vi "Main.vi"() -> ()   [LabVIEW 2013]
doc: "This template is for the Queued Message Handler design pattern.\n\nThe Event Handling Loop generates messages based on user interface actions.\n\nThe Message Handling Loop processes messages generated by the Event Handling Loop, or by other messages. The messages are string values, so new messages can be added easily to the Message Cases case structure in the Message Handling Loop. Each message cluster can also provide an optional value for Message Data, which is a variant that can be converted to whatever message-specific data is required."
uses:
  <vilib>/vision/Image Controls.llb/IMAQ Image.ctl
  Image Processing/Mask ROI FG Enum.ctl
  Message Passing/MsgQ Loops enum.ctl
  System Status/Status FG Enum.ctl
  Globals/Average Sector Data.vi
  controls/UI Data.ctl
  Message Queue/Message Queue.lvlib
  User Event - Stop/User Event - Stop.lvlib
  FPGA/FPGA Frame Grabbing.lvlib
  Image Processing/Image Processing.lvlib
  Common/State Machines/State Machine Lib.lvlib
  Message Passing/Main MsgQ.lvlib
  Common/GUI/GUI.lvlib
  <vilib>/rvi/interface/nirviReadWriteControl/nirviReadWriteControl.xnode
  FGs/FPGA_Reference.ctl
  FPGA Bitfiles/Simulation_WBA.lvbitx
  <vilib>/rvi/errors/niLvFpgaMergeErrorWithErrorCode.vi
  NiFpgaLv.dll
  <vilib>/rvi/errors/niLvFpgaAdjustHostInterfaceError.vi
panel:
  out "Frame Count":u16
  out "Frames Acquired":u32
  in  "Disable Background Subtraction":bool
  out "Analysis Ticks":u32
  out "Accumulate Ticks":u32
  out "FPGA Display Image":T1(plugin-control)
  out "Right Wingbeat Avg Graph":u8[](graph)
  in  "Start Serial Server":bool=TRUE
  out "Left Wingbeat Avg Graph":u8[](graph)
  in  "Stop Charts":bool
  in  "Wing ROIs":T2
  out "FPGA image info":T5={"Image Type"=0, "Unit"=enum."Undefined", "X Resolution"=2040, "Y Resolution"=1088, "X Step"=1.0, "Y Step"=1.0, "Image Name"="Image"} {"Image Type" items=["Grayscale (U8)", "Grayscale (I16)", "Grayscale (SGL)", "Complex (CSG)", "RGB (U32)", "HSL (U32)", "RGB (U64)", "Grayscale (U16)"]}
  in  "Stream?":bool
  out "FPGA Image":T1
  in  "Test Visual Response":bool
  in  "Test FPGA":bool
  out "Status Update":string="VI Stopped"
  in  "Define Mask":bool
  in  "Acquire Image":bool
  in  "Stop":bool
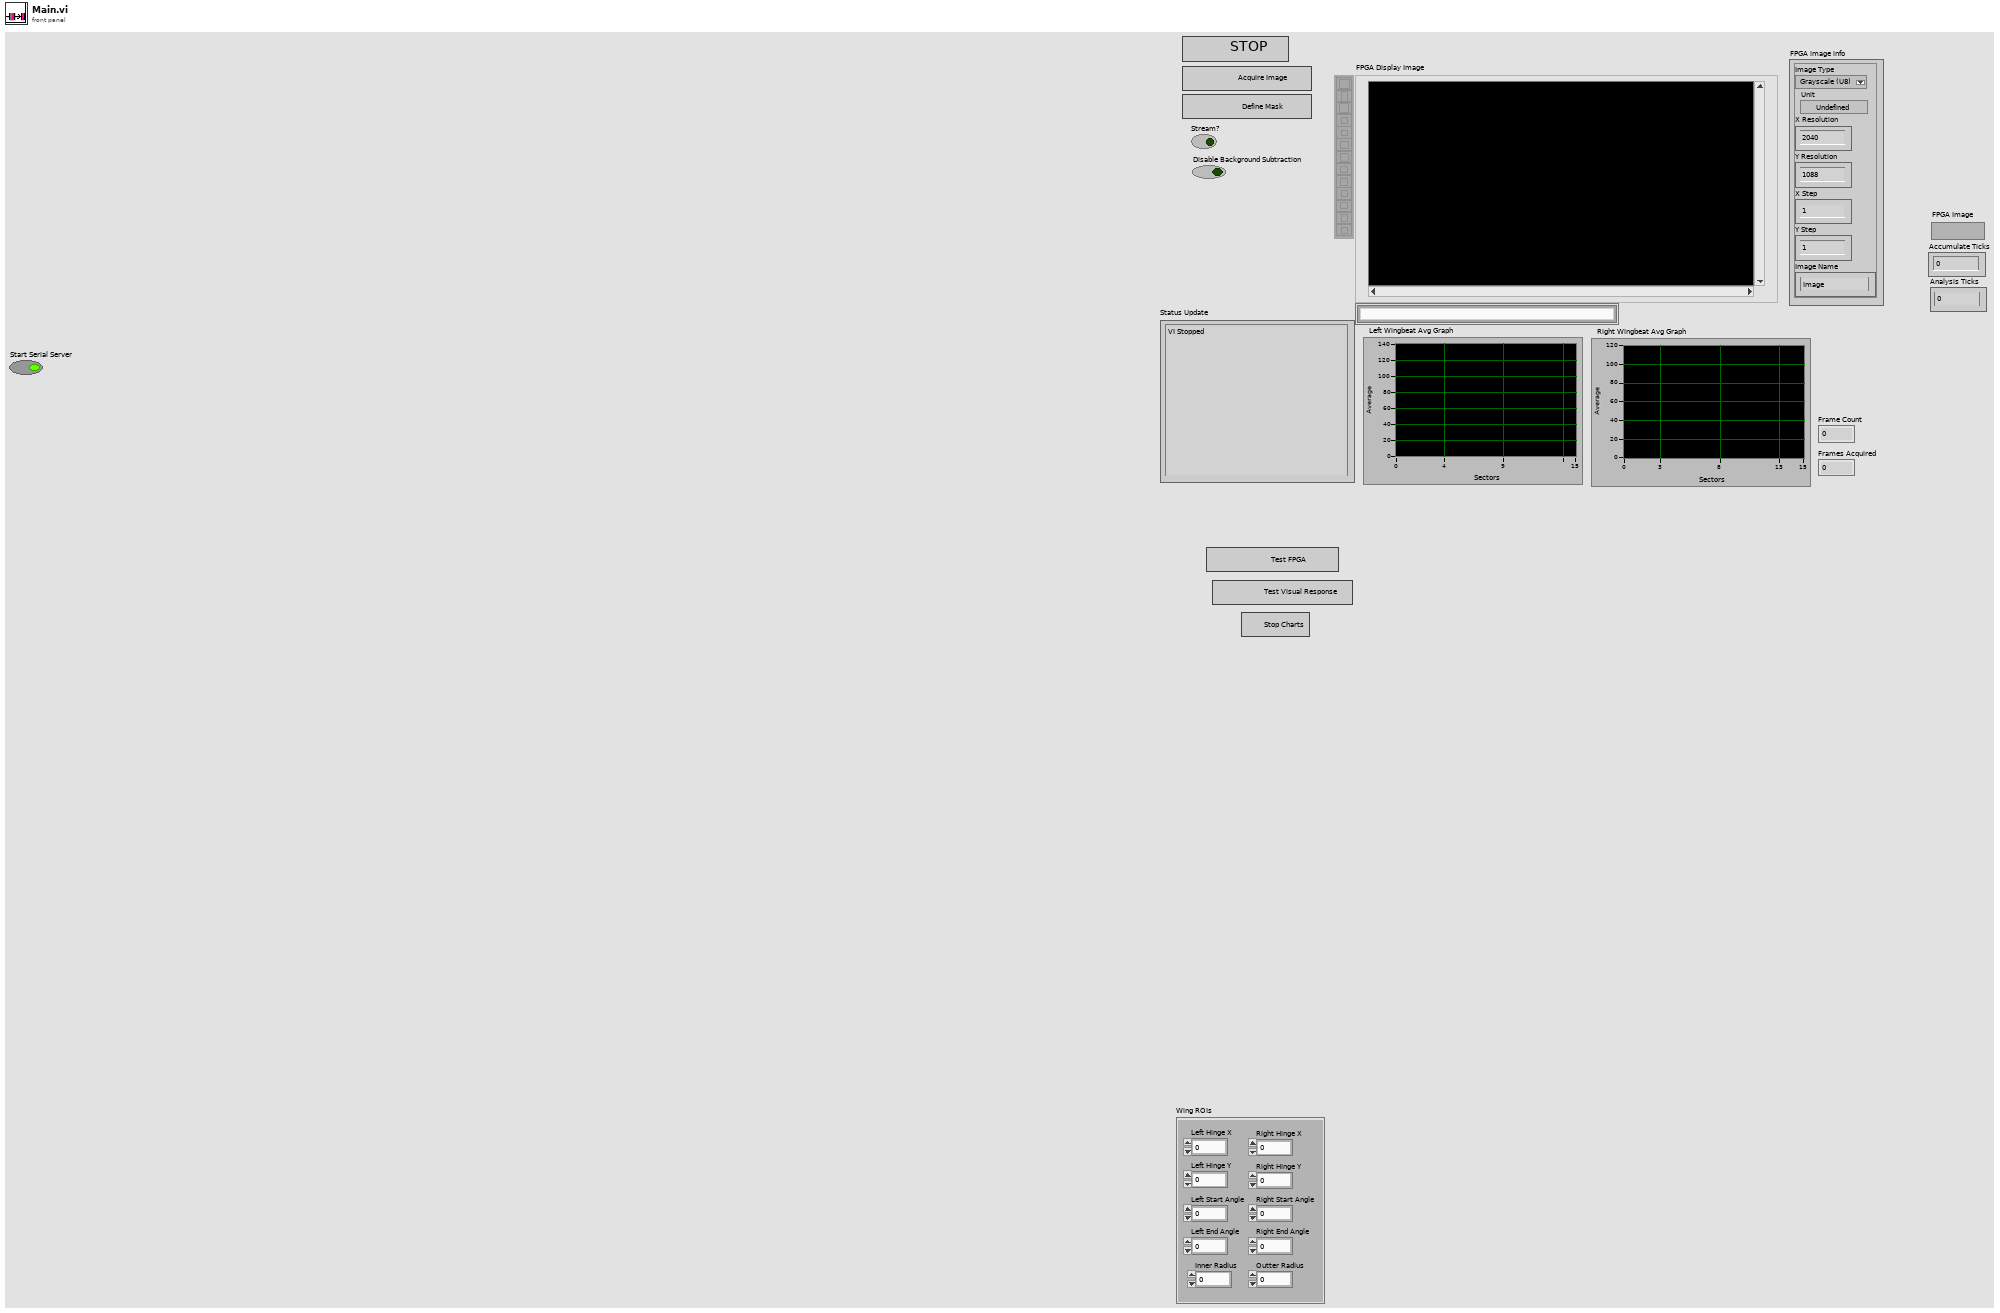
[diagram p1: front panel]
types:
  T1 = typedef "IMAQ Image.ctl" = refnum<image>
  T2 = cluster{"Left Hinge X":u16, "Left Hinge Y":u16, "Inner Radius":u16, "Outter Radius":u16, "Right Hinge X":u16, "Right Hinge Y":u16, "Right Start Angle":i16, "Right End Angle":i16, "Left Start Angle":i16, "Left End Angle":i16}
  T3 = typedef "Image Type" = u32
  T4 = typedef "Image Unit" = enum32{"Undefined", "Angström", "Micrometer", "Millimeter", "Centimeter", "Meter", "Kilometer", "Microinch", "Inch", "Feet", "Nautical miles", "Standard miles", "Steps"}
  T5 = cluster{"Image Type":T3, "Unit":T4, "X Resolution":i32, "Y Resolution":i32, "X Step":sgl, "Y Step":sgl, "Image Name":string}
  T6 = typedef "State Machine Lib.lvlib/STATE cluster.ctl" = cluster{"State":string, "Parameters":variant}
  T7 = typedef "Main MsgQ.lvlib/MsgQ Loops enum.ctl" = enum16{"User Interface", "Image Acq"}
  T8 = typedef "Mask ROI FG Enum.ctl" = enum16{"Read", "Write", "Enable Background", "Disable Background"}
  T9 = typedef "Status FG Enum.ctl" = enum16{"Reset", "Read", "Write"}
  T10 = typedef "FPGA_Reference.ctl" = refnum<k20>
  T11 = typedef "Mask ROI Cluster.ctl" = cluster{"left annulus":T12, "right annulus":T12, "Threshold Range":cluster{"Lower value":dbl, "Upper value":dbl}, "[Avg BG]":u8[], "Number of Sectors":u8, "Left ROI":T13, "Right ROI":T13, "Left Start Angle Duty Cycle":fxp<+,8,0>, "Left End Angle Duty Cycle":fxp<+,8,0>, "Right End Angle Duty Cycle":fxp<+,8,0>, "Right Start Angle Duty Cycle":fxp<+,8,0>, "[Sector ROIs]":T13[]}
  T12 = typedef "IMAQ Circle" = cluster{"Center X":i32, "Center Y":i32, "Inner Radius":i32, "Outer Radius":i32, "Start Angle":dbl, "End Angle":dbl}
  T13 = typedef "ROI Descriptor" = cluster{"Global Rectangle":i32[], "Contours":cluster{"ID":enum32{"External", "Internal"}, "Type":u32, "Coordinates":i32[]}[]}
  T14 = typedef "UI Data.ctl" = cluster{"Boolean <Replace Me>":bool, "Initial Message":string, "Numeric <Replace Me>":dbl, "Acquire Image Ref":refnum<vi>, "Define Mask Ref":refnum<vi>, "Status Update Ref":refnum<vi>, "Stop Button Ref":refnum<vi>, "FPGA Image":T1, "Processed Image":T1, "Left Annulus":cluster{"Center X":i32, "Center Y":i32, "Inner Radius":i32, "Outer Radius":i32, "Start Angle":dbl, "End Angle":dbl}, "Right Annulus":cluster{"Center X":i32, "Center Y":i32, "Inner Radius":i32, "Outer Radius":i32, "Start Angle":dbl, "End Angle":dbl}}
  T15 = typedef "Message Queue.lvlib/All Message Queues.ctl" = cluster{"UI":refnum<queue>}
  T16 = cluster{"Center X":i32, "Center Y":i32, "Inner Radius":i32, "Outer Radius":i32, "Start Angle":dbl, "End Angle":dbl}
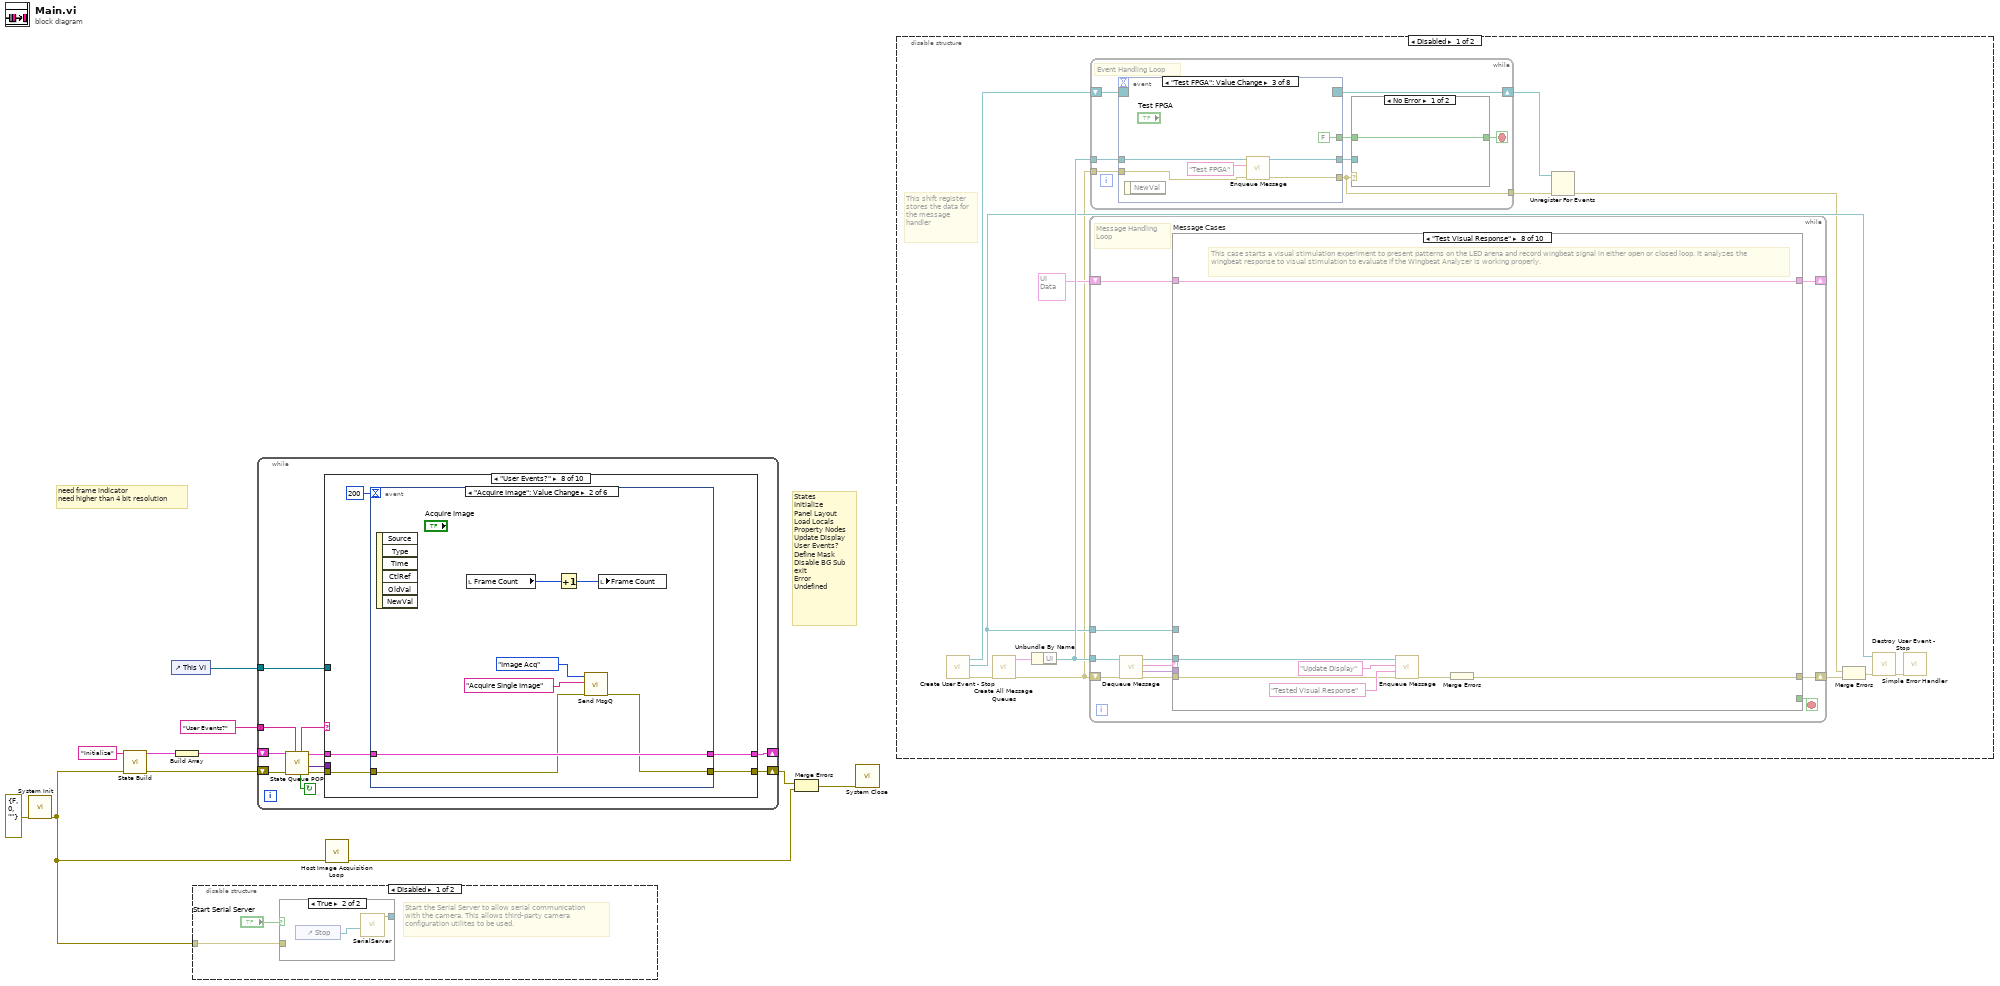
[diagram p0: block diagram]
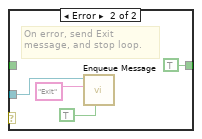
[diagram p4: hidden frame]
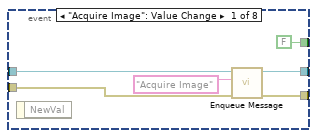
[diagram p5: hidden frame]
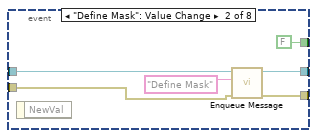
[diagram p6: hidden frame]
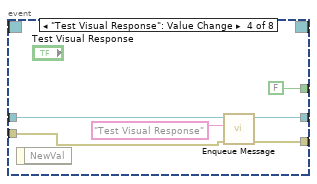
[diagram p7: hidden frame]
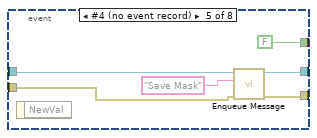
[diagram p8: hidden frame]
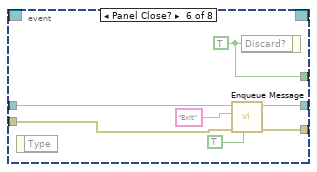
[diagram p9: hidden frame]
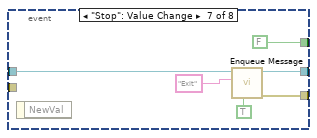
[diagram p10: hidden frame]
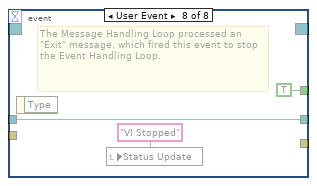
[diagram p11: hidden frame]
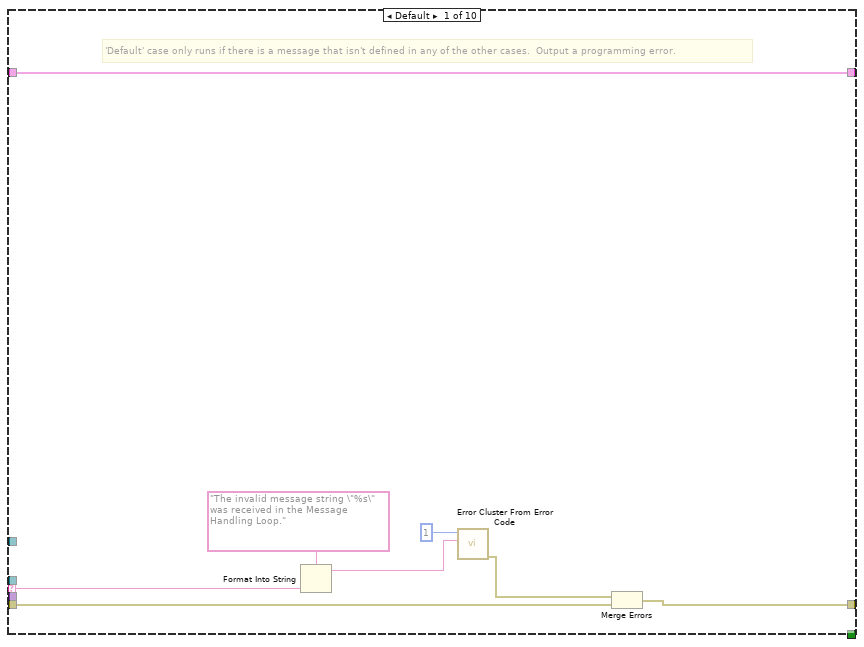
[diagram p12: hidden frame]
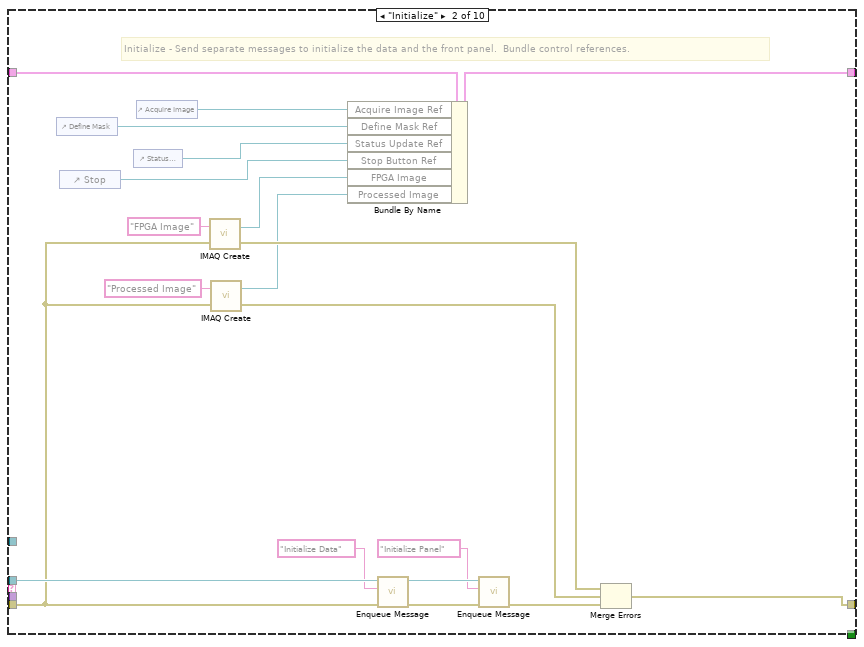
[diagram p13: hidden frame]
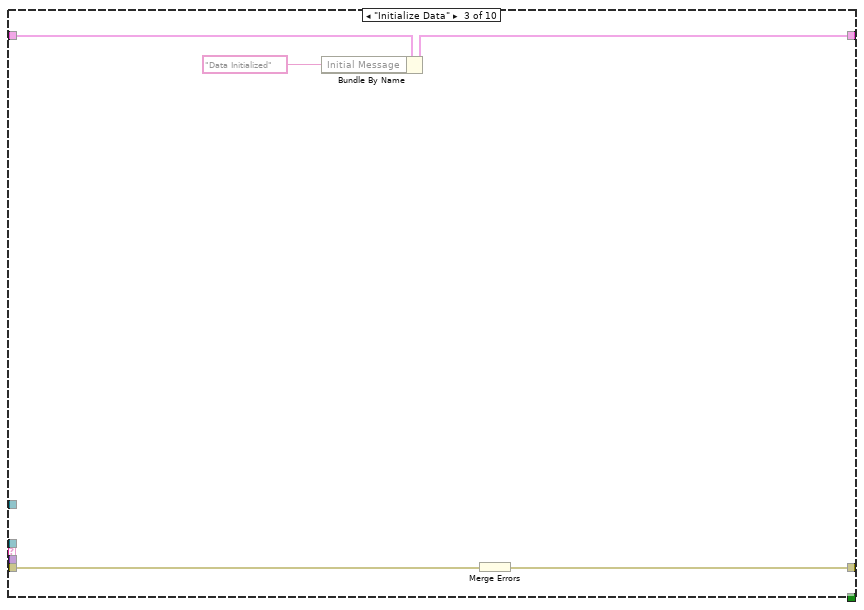
[diagram p14: hidden frame]
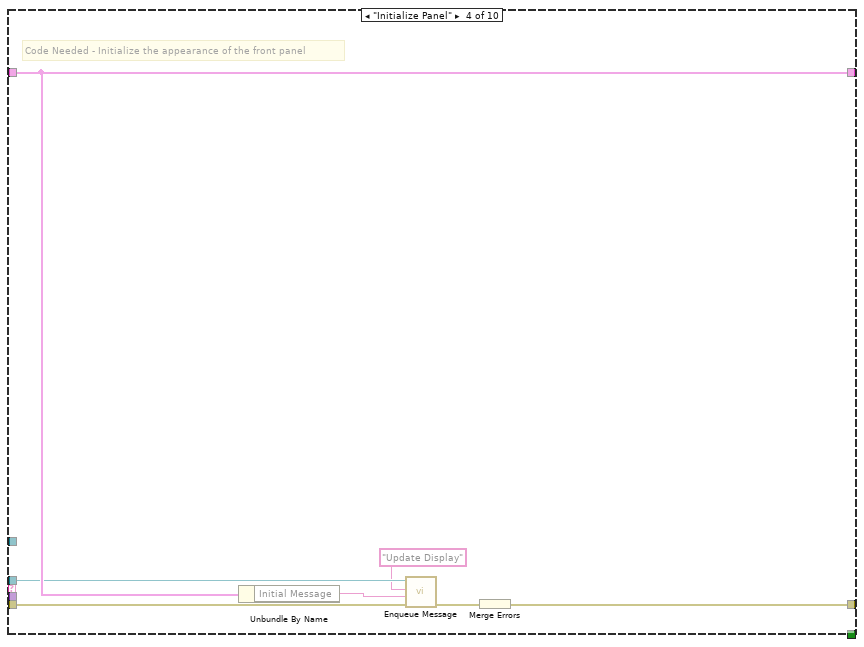
[diagram p15: hidden frame]
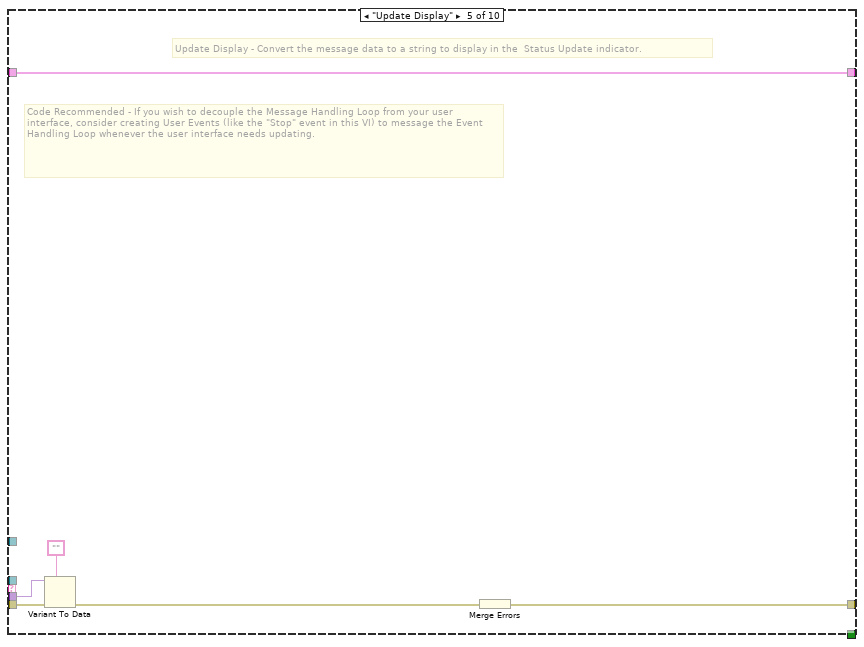
[diagram p16: hidden frame]
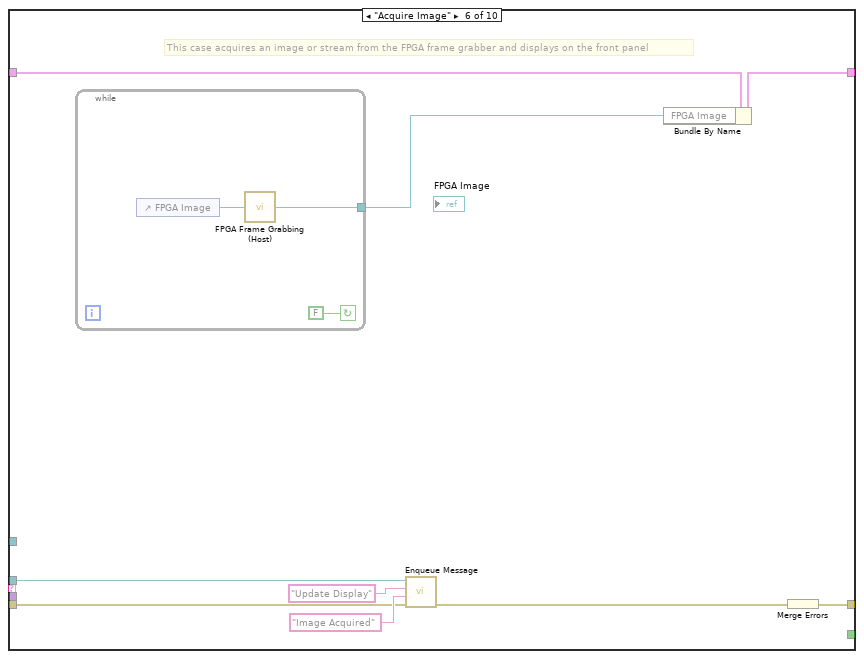
[diagram p17: hidden frame]
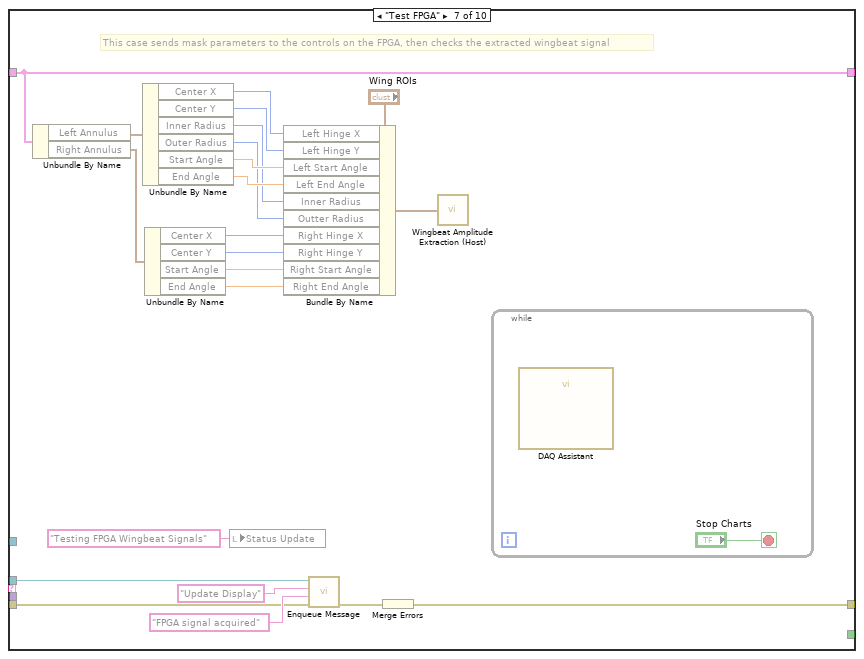
[diagram p18: hidden frame]
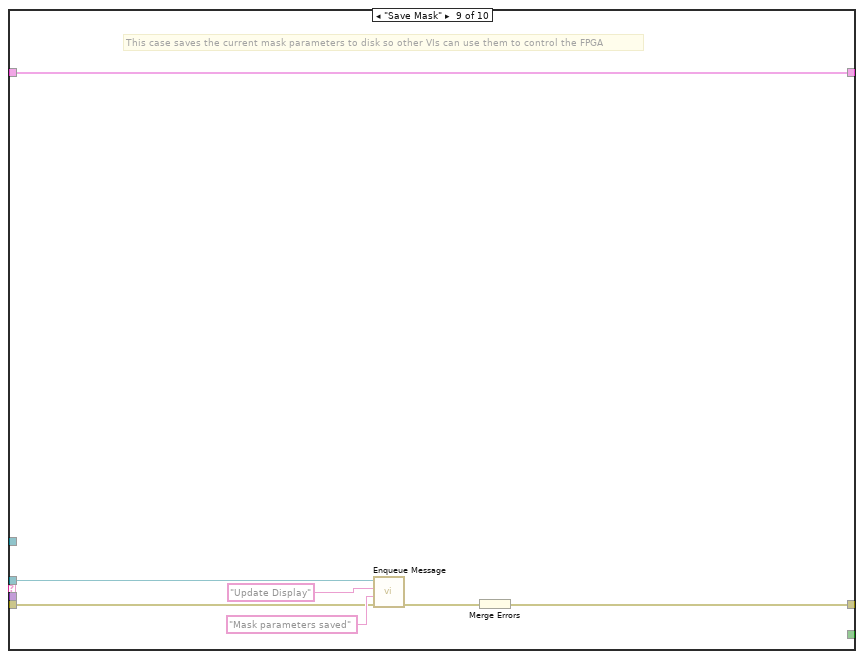
[diagram p19: hidden frame]
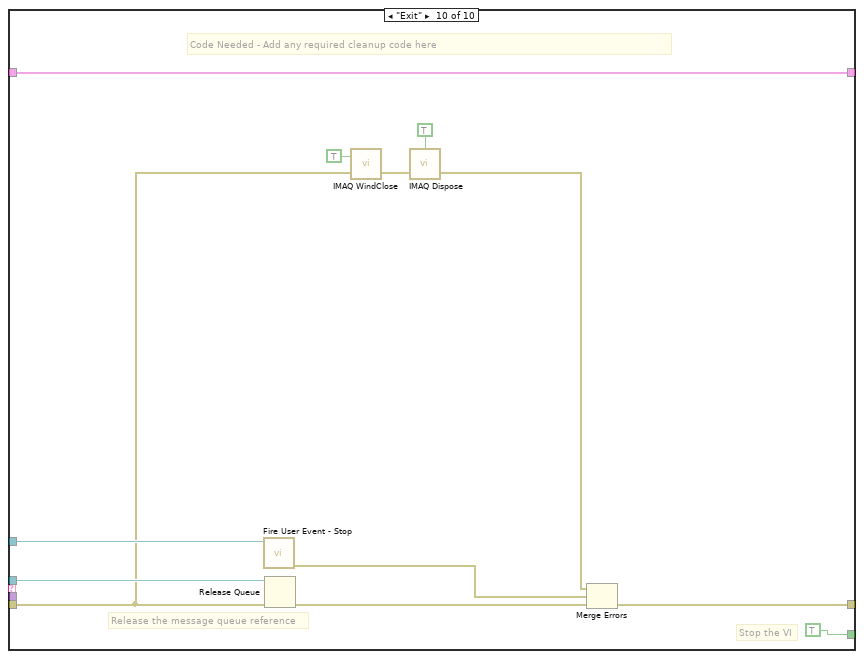
[diagram p20: hidden frame]
diagram:
  # "need frame indicator\nneed higher than 4 bit resolution"
  # "States\nInitialize\nPanel Layout\nLoad Locals\nProperty Nodes\nUpdate Display\nUser Events?\nDefine Mask\nDisable BG Sub\nexit\nError\nUndefined"
  n1 = call "System Init.vi"("error in (no error)"=errorcluster {"status"=FALSE, "code"=0, "source"=""}) -> ("error out"=w10:errorcluster)  [unwired: 10 in]
  n2 = call "State Build.vi"("error in (no error)"=w10, "State"="Initialize") -> ("error out"=w6:errorcluster, "State Out"=w8:T6)  [unwired: 8 in]
  n3 = control-ref of="This VI"() -> (w4:refnum<vi>)
  n4 = Build Array(w8) -> (w7:T6[])
  n5 = disable-structure shown="Disabled" {
    disable-tunnel: w10 -> [w12 _]
    frame Disabled {
      # "Start the Serial Server to allow serial communication\nwith the camera. This allows third-party camera\nconfiguration utilites to be used."
      n6 = case shown="True" "Start Serial Server" {
        tunnel: [_ w15] -> _
        tunnel: w12 -> [_ _]
        frame False {
        }
        frame True {
          n7 = control-ref of="Stop"() -> (w14:refnum<vi>)
          n8 = call "SerialServer.vi"("Stop Refnum"=w14) -> ("FPGA VI Reference Out"=w15:refnum<k20>)  [unwired: 6 in]
        }
      }
    }
    frame Enabled {
    }
  }
  n9 = while {
    shift-right: [w20] -> _
    shift-left: w7 -> [w26]
    shift-right: [w18] -> w3
    shift-left: w6 -> [w25]
    tunnel: "User Events?" ("State") -> [w23]
    tunnel: w4 -> [w21]
    stop <- w24 continue-if-true
    n10 = call "State Queue POP.vi"("Default state"=w23, "error in (no error)"=w25, "State que in"=w26) -> ("error out"=w17:errorcluster, "Parameters"=w16:variant, "State que out"=w19:T6[], "Not Exit?"=w24:bool, "State case out"=w22:string)  [unwired: 4 in]
    n11 = case shown="\"User Events?\"" w22 {
      tunnel: w21 -> [_ _ w37 _ _ _ _ _ _ _]
      tunnel: [w28 w29 w34 w41 w43 w48 w49 w65 w105 w133] -> w20
      tunnel: w19 -> [w28 w32 w34 w41 w43 w48 w49 w64 _ w133]
      tunnel: [w27 w30 w35 w40 w42 w46 w50 w63 w104 w131] -> w18
      tunnel: w17 -> [w27 w31 w36 w40 w42 w47 w51 w62 w106 w115]
      tunnel: w16 -> [_ _ _ _ _ _ w52 _ _ _]
      frame Default {
      }
      frame "Initialize" {
        n12 = call "State Queue PUSH multiple states no parameters.vi"("States to queue"=string[] ["Panel Layout", "Load Locals", "Property Nodes", "Update Display"], "error in (no error)"=w31, "State que in"=w32) -> ("error out"=w30:errorcluster, "State que out"=w29:T6[])  [unwired: 7 in]
      }
      frame "Panel Layout" {
        # "Reset origin to 0,0"
        n13 = call "Reset all pane origins.vi"("error in (no error"=w36, "Vi Ref In"=w37) -> ("error out"=w35:errorcluster)  [unwired: 8 in, 1 out]
      }
      frame "Load Locals" {
        w39 = FALSE ("Stream?")
        n14 = local write "Stream?"(w39) -> ()
        n15 = local write "Disable Background Subtraction"(w39) -> ()
        "Frame Count" <- u16 0 ("Frame Count")
      }
      frame "Property Nodes" {
      }
      frame "Define Mask" {
        n16 = call "Image References.vi"() -> ("Images"=w44:cluster{"Acquired Image":T1, "Display Image":T1})  [unwired: 10 in, 1 out]
        n17 = Unbundle By Name(w44) -> ("Acquired Image"=w45:T1)
        n18 = call "Define Mask.vi"("error in (no error)"=w47, "FPGA Image"=w45) -> ("error out"=w46:errorcluster)  [unwired: 9 in]
      }
      frame "Disable BG Sub" {
        n19 = Variant To Data(error in=w51, type=FALSE, Variant=w52) -> (data=w60:bool, error out=w57:errorcluster)
        n20 = Select(t=Mask_ROI_FG_Enum."Disable Background" ("Operation"), s=w60, f=Mask_ROI_FG_Enum."Enable Background" ("Operation")) -> (s? t:f=w56:T8)
        n21 = call "Mask ROI FG.vi"("error in (no error)"=w57, "Operation"=w56) -> ("error out"=w53:errorcluster)  [unwired: 8 in, 1 out]
        n22 = call "Send MsgQ.vi"("error in (no error)"=w53, "Message String"="Update Sector Parameters", "Send to MsgQ"=MsgQ_Loops_enum."Image Acq") -> ("error out"=w50:errorcluster)  [unwired: 8 in]
      }
      frame "User Events?" {
        n23 = event shown="[1] \"Acquire Image\": Value Change" {
          selector: _ -> [_ _ _ _ _ _]
          dyn-events: _ -> [_ _ _ _ _ _]
          timeout: 200 -> [_ _ _ _ _ _]
          tunnel: [w68 w80 w83 w90 w96 w99] -> w65
          tunnel: w64 -> [w69 w80 w83 w92 w97 w102]
          tunnel: [w70 w77 w84 w89 w95 w100] -> w63
          tunnel: w62 -> [w71 w78 w85 w91 w94 w101]
          event Timeout {
            n24 = event-data() -> ()  [unwired: 1 in, 3 out]
            n25 = disable-structure shown="Disabled" {
              frame Disabled {
                n26 = call "FPGA Reference FG.vi"() -> ("FPGA VI Reference Out"=w74:T10)  [unwired: 11 in]
                n27 = xnode "Read/Write Control"("FPGA VI Reference In"=w74) -> ("Accumulate Ticks"=→"Accumulate Ticks", "Analysis Ticks"=→"Analysis Ticks":u32)  [unwired: 1 in, 2 out]
              }
              frame Enabled {
              }
            }
            n28 = call "State Queue PUSH.vi"("State case"="Update Display", "error in (no error)"=w71, "State que in"=w69) -> ("error out"=w70:errorcluster, "State que out"=w68:T6[])  [unwired: 7 in]
          }
          event "Acquire Image": Value Change {
            n29 = event-data() -> ()  [unwired: 1 in, 6 out]
            n30 = local read "Frame Count"() -> (w76:u16)
            n31 = Increment(x=w76) -> (x+1=w75:u16)
            n32 = call "Send MsgQ.vi"("error in (no error)"=w78, "Message String"="Acquire Single Image", "Send to MsgQ"=MsgQ_Loops_enum."Image Acq") -> ("error out"=w77:errorcluster)  [unwired: 8 in]
            n33 = local write "Frame Count"(w75) -> ()
          }
          event "Stream?": Value Change {
            n34 = event-data() -> ("NewVal"=w82:bool)  [unwired: 1 in, 5 out]
            n35 = call "Send MsgQ.vi"("error in (no error)"=w85, "Data In"=w82, "Message String"="Stream Image", "Send to MsgQ"=MsgQ_Loops_enum."Image Acq") -> ("error out"=w84:errorcluster)  [unwired: 7 in]
          }
          event "Define Mask": Value Change {
            n36 = event-data() -> ()  [unwired: 1 in, 6 out]
            n37 = call "State Queue PUSH.vi"("State case"="Define Mask", "error in (no error)"=w91, "State que in"=w92) -> ("error out"=w89:errorcluster, "State que out"=w90:T6[])  [unwired: 7 in]
          }
          event "Disable Background Subtraction": Value Change {
            n38 = event-data() -> ("NewVal"=w93:bool)  [unwired: 1 in, 5 out]
            n39 = call "State Queue PUSH.vi"("State case"="Disable BG Sub", "error in (no error)"=w94, "Parameters"=w93, "State que in"=w97) -> ("error out"=w95:errorcluster, "State que out"=w96:T6[])  [unwired: 6 in]
          }
          event "Stop": Value Change {
            n40 = event-data() -> ()  [unwired: 1 in, 6 out]
            n41 = call "State Queue PUSH.vi"("State case"="exit", "error in (no error)"=w101, "State que in"=w102) -> ("error out"=w100:errorcluster, "State que out"=w99:T6[])  [unwired: 7 in]
          }
        }
      }
      frame "exit" {
        n42 = call "Broadcast Exit.vi"("error in"=w106) -> ("error out"=w104:errorcluster)  [unwired: 10 in]
        n43 = call "Queue EXIT state.vi"() -> ("Exit State Q"=w105:T6[])  [unwired: 1 in]
      }
      frame "Update Display" {
        n44 = global read "Average Sector Data.vi" "# of Frames Acquired"() -> (→"Frames Acquired":u32)
        n45 = call "Image References.vi"() -> ("Images"=w111:cluster{"Acquired Image":T1, "Display Image":T1})  [unwired: 10 in, 1 out]
        n46 = call "Status FG.vi"("Operation"=Status_FG_Enum."Read") -> ("Status Out"=→"Status Update":string)  [unwired: 9 in, 1 out]
        n47 = call "Mask ROI FG.vi"("Operation"=Mask_ROI_FG_Enum."Read") -> ("Mask ROI Out"=w128:T11)  [unwired: 9 in, 1 out]
        n48 = Unbundle By Name(w111) -> ("Acquired Image"=w110:T1, "Display Image"=w109:T1)
        n49 = Unbundle By Name(w128) -> ("Number of Sectors"=w125:u8)
        n50 = global read "Average Sector Data.vi" "[Average Sector Data]"() -> (w130:u8[])
        n51 = call "Overlay Image with Sector ROI.vi"("FPGA Display Image In"=w109, "error in"=w115, "FPGA Image"=w110) -> ("error out"=w114:errorcluster, "FPGA Display Image Out"=→"FPGA Display Image":T1)  [unwired: 7 in]
        n52 = call "IMAQ GetImageInfo"("error in (no error)"=w114, "Image"=w110) -> ("error out"=w132:errorcluster, "X Step"=w120:sgl, "Y Resolution"=w119:i32, "X Resolution"=w118:i32, "Y Step"=w121:sgl, "Unit"=w117:T4, "Image Name"=w122:string, "Image Type"=w116:T3)  [unwired: 2 in]
        n53 = Split 1D Array(array=w130, index=w125) -> (first subarray=→"Left Wingbeat Avg Graph":u8[], second subarray=→"Right Wingbeat Avg Graph":u8[])
        n54 = local read "FPGA image info"() -> (w124:T5)
        n55 = Bundle By Name(cluster=w124, "Image Type"=w116, "Unit"=w117, "X Resolution"=w118, "Y Resolution"=w119, "X Step"=w120, "Y Step"=w121, "Image Name"=w122) -> (→"FPGA image info":T5)
        n56 = call <vilib>:"Clear Errors.vi"("error in (no error)"=w132) -> ("error out"=w131:errorcluster)  [unwired: 6 in]
      }
    }
  }
  n57 = call "Host Image Acquisition Loop.vi"("error in"=w10) -> ("error out"=w2:errorcluster)  [unwired: 10 in]
  n58 = Merge Errors(w3, w2) -> (w1:errorcluster)
  n59 = call "System Close.vi"("error in (no error)"=w1) -> ()  [unwired: 10 in, 1 out]
  n60 = disable-structure shown="Disabled" {
    frame Disabled {
      # "This shift register\nstores the data for the message handler"
      n61 = call "Create User Event - Stop.vi"() -> ("error out"=w142:errorcluster, "User Event - Stop"=w139:refnum<user-event>, "Stop Event Registration Refnum"=w143:refnum<event-registration>)  [unwired: 9 in]
      n62 = call "Create All Message Queues.vi"("error in (no error)"=w142) -> ("error out"=w134:errorcluster, "Message Queues out"=w146:T15)  [unwired: 9 in]
      n63 = Unbundle By Name(w146) -> ("UI"=w144:refnum<queue>)
      n64 = while {
        tunnel: w144 -> [w206]
        shift-right: [w215] -> _
        shift-left: T14 {"Boolean <Replace Me>"=TRUE, "Initial Message"="", "Numeric <Replace Me>"=0.0, "Acquire Image Ref"=refnum, "Define Mask Ref"=refnum, "Status Update Ref"=refnum, "Stop Button Ref"=refnum, "FPGA Image"=refnum, "Processed Image"=refnum, "Left Annulus"={"Center X"=0, "Center Y"=0, "Inner Radius"=0, "Outer Radius"=0, "Start Angle"=0.0, "End Angle"=0.0}, "Right Annulus"={"Center X"=0, "Center Y"=0, "Inner Radius"=0, "Outer Radius"=0, "Start Angle"=0.0, "End Angle"=0.0}} ("Data Cluster") -> [w216]
        tunnel: w139 -> [w212]
        shift-right: [w213] -> w145
        shift-left: w134 -> [w211]
        stop <- w214 stop-if-true
        # "Message Handling Loop"
        n65 = call "Dequeue Message.vi"("error in (no error)"=w211, "Message Queue"=w206) -> ("error out"=w210:errorcluster, "Message Data"=w208:variant, "Message"=w209:string, "dup Message Queue"=w207:refnum<queue>)  [unwired: 6 in]
        n66 = case "Message Cases" shown="\"Test Visual Response\"" w209 {
          selector: w209 -> [w222 _ _ _ _ _ _ _ _ _]
          tunnel: w207 -> [_ w242 _ w253 _ w270 w293 w301 w309 w325]
          tunnel: w210 -> [w219 w227 w249 w254 w261 w265 w294 w302 w307 w314]
          tunnel: [w217 w229 w245 w255 w262 w272 w292 w300 w312 w321] -> w213
          tunnel: w216 -> [w224 w239 w248 w256 w263 w267 w291 w306 w313 w324]
          tunnel: [w224 w238 w247 w256 w263 w266 w291 w306 w313 w324] -> w215
          tunnel: [_ _ _ _ _ _ _ _ _ TRUE] -> w214
          tunnel: w208 -> [_ _ _ _ w260 _ _ _ _ _]
          tunnel: w212 -> [_ _ _ _ _ _ _ _ _ w320]
          frame Default {
            # "'Default' case only runs if there is a message that isn't defined in any of the other cases.  Output a programming error."
            n67 = Format Into String(format string="The invalid message string \"%s\" was received in the Message Handling Loop." ("Unknown Message Error Text"), w222) -> (resulting string=w220:string)  [unwired: 2 in, 1 out]
            n68 = call <vilib>:"Error Cluster From Error Code.vi"("error message (\"\")"=w220, "error code (0)"=1) -> ("error out"=w218:errorcluster)  [unwired: 7 in]
            n69 = Merge Errors(w218, w219) -> (w217:errorcluster)
          }
          frame "Initialize" {
            # "Initialize - Send separate messages to initialize the data and the front panel.  Bundle control references."
            n70 = control-ref of="Define Mask"() -> (w236:refnum<vi>)
            n71 = control-ref of="Stop"() -> (w234:refnum<vi>)
            n72 = control-ref of="Status Update"() -> (w235:refnum<vi>)
            n73 = control-ref of="Acquire Image"() -> (w237:refnum<vi>)
            n74 = call "IMAQ Create"("Image Name"="FPGA Image", "error in (no error)"=w227) -> ("New Image"=w232:T1, "error out"=w228:errorcluster)  [unwired: 3 in]
            n75 = call "IMAQ Create"("Image Name"="Processed Image", "error in (no error)"=w227) -> ("New Image"=w225:T1, "error out"=w226:errorcluster)  [unwired: 3 in]
            n76 = Bundle By Name(cluster=w239, "Acquire Image Ref"=w237, "Define Mask Ref"=w236, "Status Update Ref"=w235, "Stop Button Ref"=w234, "FPGA Image"=w232, "Processed Image"=w225) -> (w238:T14)
            n77 = call "Enqueue Message.vi"("error in (no error)"=w227, "Message"="Initialize Data", "Message Queue"=w242) -> ("error out"=w244:errorcluster, "dup Message Queue"=w243:refnum<queue>)  [unwired: 7 in]
            n78 = call "Enqueue Message.vi"("error in (no error)"=w244, "Message"="Initialize Panel", "Message Queue"=w243) -> ("error out"=w230:errorcluster)  [unwired: 7 in, 1 out]
            n79 = Merge Errors(w228, w226, w230) -> (w229:errorcluster)
          }
          frame "Initialize Data" {
            n80 = Bundle By Name(cluster=w248, "Initial Message"="Data Initialized") -> (w247:T14)
            n81 = Merge Errors(w249) -> (w245:errorcluster)
          }
          frame "Initialize Panel" {
            # "Code Needed - Initialize the appearance of the front panel"
            n82 = Unbundle By Name(w256) -> ("Initial Message"=w250:string)
            n83 = call "Enqueue Message.vi"("error in (no error)"=w254, "Message Data"=w250, "Message"="Update Display", "Message Queue"=w253) -> ("error out"=w252:errorcluster)  [unwired: 6 in, 1 out]
            n84 = Merge Errors(w252) -> (w255:errorcluster)
          }
          frame "Update Display" {
            # "Code Recommended - If you wish to decouple the Message Handling Loop from your user interface, consider creating User Events (like the \"Stop\" event in this VI) to message the Event Handling Loop whenever the user interface needs updating."
            # "Update Display - Convert the message data to a string to display in the  Status Update indicator."
            n85 = Variant To Data(error in=w261, type="", Variant=w260) -> (data=w257:string, error out=w258:errorcluster)
            n86 = Merge Errors(w258) -> (w262:errorcluster)
          }
          frame "Acquire Image" {
            # "This case acquires an image or stream from the FPGA frame grabber and displays on the front panel"
            n87 = while {
              tunnel: [w275] -> w264
              stop <- FALSE continue-if-true
              n88 = control-ref of="FPGA Image"() -> (w274:refnum<vi>)
              n89 = call "FPGA Frame Grabbing (Host).vi"("Ctl Refnum"=w274) -> ("Image"=w275:T1)
            }
            n90 = call "Enqueue Message.vi"("error in (no error)"=w265, "Message Data"="Image Acquired" ("\"Do Something\" button pressed"), "Message"="Update Display", "Message Queue"=w270) -> ("error out"=w271:errorcluster)  [unwired: 6 in, 1 out]
            n91 = Bundle By Name(cluster=w267, "FPGA Image"=w264) -> (w266:T14)
            n92 = Merge Errors(w271) -> (w272:errorcluster)
          }
          frame "Test FPGA" {
            # "This case sends mask parameters to the controls on the FPGA, then checks the extracted wingbeat signal"
            n93 = Unbundle By Name(w291) -> ("Left Annulus"=w290:T16, "Right Annulus"=w289:T16)
            n94 = Unbundle By Name(w290) -> ("Center X"=w287:i32, "Center Y"=w286:i32, "Inner Radius"=w283:i32, "Outer Radius"=w282:i32, "Start Angle"=w285:dbl, "End Angle"=w284:dbl)
            n95 = Unbundle By Name(w289) -> ("Center X"=w281:i32, "Center Y"=w280:i32, "Start Angle"=w279:dbl, "End Angle"=w278:dbl)
            n96 = local write "Status Update"("Testing FPGA Wingbeat Signals" ("Status Update")) -> ()
            n97 = Bundle By Name(cluster="Wing ROIs", "Left Hinge X"=w287, "Left Hinge Y"=w286, "Left Start Angle"=w285, "Left End Angle"=w284, "Inner Radius"=w283, "Outter Radius"=w282, "Right Hinge X"=w281, "Right Hinge Y"=w280, "Right Start Angle"=w279, "Right End Angle"=w278) -> (w277:T2)
            n98 = call "Enqueue Message.vi"("error in (no error)"=w294, "Message Data"="FPGA signal acquired" ("\"Do Something\" button pressed"), "Message"="Update Display", "Message Queue"=w293) -> ("error out"=w297:errorcluster)  [unwired: 6 in, 1 out]
            n99 = Merge Errors(w297) -> (w292:errorcluster)
            n100 = call "Wingbeat Amplitude Extraction (Host).vi"("Wing ROIs"=w277) -> ()  [unwired: 1 in]
            n101 = while {
              stop <- "Stop Charts" stop-if-true
              n102 = call "DAQ Assistant"() -> ("data"=w298:dynamicdata)  [unwired: 17 in, 2 out]
            }
          }
          frame "Test Visual Response" {
            # "This case starts a visual stimulation experiment to present patterns on the LED arena and record wingbeat signal in either open or closed loop. It analyzes the wingbeat response to visual stimulation to evaluate if the Wingbeat Analyzer is working properly."
            n103 = call "Enqueue Message.vi"("error in (no error)"=w302, "Message Data"="Tested Visual Response" ("\"Do Something\" button pressed"), "Message"="Update Display", "Message Queue"=w301) -> ("error out"=w305:errorcluster)  [unwired: 6 in, 1 out]
            n104 = Merge Errors(w305) -> (w300:errorcluster)
          }
          frame "Save Mask" {
            # "This case saves the current mask parameters to disk so other VIs can use them to control the FPGA"
            n105 = call "Enqueue Message.vi"("error in (no error)"=w307, "Message Data"="Mask parameters saved" ("\"Do Something Else\" button pressed"), "Message"="Update Display", "Message Queue"=w309) -> ("error out"=w308:errorcluster)  [unwired: 6 in, 1 out]
            n106 = Merge Errors(w308) -> (w312:errorcluster)
          }
          frame "Exit" {
            # "Stop the VI"
            # "Release the message queue reference"
            # "Code Needed - Add any required cleanup code here"
            n107 = call "Fire User Event - Stop.vi"("User Event - Stop"=w320) -> ("error out"=w319:errorcluster)  [unwired: 10 in]
            n108 = Release Queue(queue=w325, error in (no error)=w314) -> (error out=w322:errorcluster)  [unwired: 1 in, 2 out]
            n109 = call "IMAQ WindClose"("Close All Windows (False)"=TRUE, "error in (no error)"=w314) -> ("error out"=w316:errorcluster)  [unwired: 4 in]
            n110 = call "IMAQ Dispose"("All Images? (No)"=TRUE, "error in (no error)"=w316) -> ("error out"=w315:errorcluster)  [unwired: 4 in]
            n111 = Merge Errors(w315, w319, w322) -> (w321:errorcluster)
          }
        }
      }
      n112 = while {
        tunnel: w144 -> [w154]
        tunnel: [w150] -> w137
        shift-right: [w148] -> w136
        shift-left: w143 -> [w149]
        tunnel: w134 -> [w147]
        stop <- w152 stop-if-true
        # "Event Handling Loop"
        n113 = event shown="[2] \"Test FPGA\": Value Change" {
          selector: w149 -> [_ _ _ _ _ _ _ _]
          dyn-events: [_ _ _ _ _ _ _ _] -> w148
          timeout: _ -> [_ _ _ _ _ _ _ _]
          tunnel: [FALSE ("Discard?") FALSE ("Discard?") FALSE ("Discard?") FALSE ("Discard?") FALSE ("Discard?") w196 FALSE ("Discard?") TRUE ("Discard?")] -> w153
          tunnel: w154 -> [w165 w171 w177 w182 w187 w195 w202 w205]
          tunnel: [w164 w169 w174 w179 w184 w194 w201 _] -> w150
          tunnel: [w163 w170 w173 w181 w186 w193 w199 w205] -> w151
          tunnel: w147 -> [w161 w167 w175 w178 w185 w190 _ _]
          event "Acquire Image": Value Change {
            n114 = event-data() -> ()  [unwired: 1 in, 1 out]
            n115 = call "Enqueue Message.vi"("error in (no error)"=w161, "Message"="Acquire Image", "Message Queue"=w165) -> ("error out"=w164:errorcluster, "dup Message Queue"=w163:refnum<queue>)  [unwired: 7 in]
          }
          event "Define Mask": Value Change {
            n116 = event-data() -> ()  [unwired: 1 in, 1 out]
            n117 = call "Enqueue Message.vi"("error in (no error)"=w167, "Message"="Define Mask", "Message Queue"=w171) -> ("error out"=w169:errorcluster, "dup Message Queue"=w170:refnum<queue>)  [unwired: 7 in]
          }
          event "Test FPGA": Value Change {
            n118 = event-data() -> ()  [unwired: 1 in, 1 out]
            n119 = call "Enqueue Message.vi"("error in (no error)"=w175, "Message"="Test FPGA", "Message Queue"=w177) -> ("error out"=w174:errorcluster, "dup Message Queue"=w173:refnum<queue>)  [unwired: 7 in]
          }
          event "Test Visual Response": Value Change {
            n120 = event-data() -> ()  [unwired: 1 in, 1 out]
            n121 = call "Enqueue Message.vi"("error in (no error)"=w178, "Message"="Test Visual Response", "Message Queue"=w182) -> ("error out"=w179:errorcluster, "dup Message Queue"=w181:refnum<queue>)  [unwired: 7 in]
          }
          event #4 (no event record) {
            n122 = event-data() -> ()  [unwired: 1 in, 1 out]
            n123 = call "Enqueue Message.vi"("error in (no error)"=w185, "Message"="Save Mask", "Message Queue"=w187) -> ("error out"=w184:errorcluster, "dup Message Queue"=w186:refnum<queue>)  [unwired: 7 in]
          }
          event Panel Close? {
            w196 = TRUE ("Discard?")
            n124 = event-data() -> ()  [unwired: 1 in, 1 out]
            n125 = call "Enqueue Message.vi"("Priority Message? (F)"=TRUE, "error in (no error)"=w190, "Message"="Exit", "Message Queue"=w195) -> ("error out"=w194:errorcluster, "dup Message Queue"=w193:refnum<queue>)  [unwired: 6 in]
            n126 = event-data("Discard?"=w196) -> ()  [unwired: 1 in, 1 out]
          }
          event "Stop": Value Change {
            n127 = event-data() -> ()  [unwired: 1 in, 1 out]
            n128 = call "Enqueue Message.vi"("Priority Message? (F)"=TRUE, "Message"="Exit", "Message Queue"=w202) -> ("error out"=w201:errorcluster, "dup Message Queue"=w199:refnum<queue>)  [unwired: 7 in]
          }
          event User Event {
            # "The Message Handling Loop processed an \"Exit\" message, which fired this event to stop the Event Handling Loop."
            n129 = event-data() -> ()  [unwired: 1 in, 1 out]
            n130 = local write "Status Update"("VI Stopped" ("VI Stopped")) -> ()
          }
        }
        n131 = case shown="No Error" w150 {
          tunnel: [w155 TRUE ("Discard?")] -> w152
          tunnel: w153 -> [w155 _]
          tunnel: w151 -> [_ w158]
          frame No Error {
          }
          frame Error {
            # "On error, send Exit message, and stop loop."
            n132 = call "Enqueue Message.vi"("Priority Message? (F)"=TRUE, "Message"="Exit", "Message Queue"=w158) -> ()  [unwired: 7 in, 2 out]
          }
        }
      }
      n133 = Unregister For Events(event registration refnum=w136, error in=w137) -> (error out=w138:errorcluster)
      n134 = Merge Errors(w138, w145) -> (w140:errorcluster)
      n135 = call "Destroy User Event - Stop.vi"("error in (no error)"=w140, "User Event - Stop"=w139) -> ("error out"=w141:errorcluster)  [unwired: 9 in]
      n136 = call <vilib>:"Simple Error Handler.vi"("error in (no error)"=w141) -> ()  [unwired: 4 in, 5 out]
    }
    frame Enabled {
    }
  }
